vi "Ecrire config.vi"(2 "error in (no error)":errorcluster caption="entrée d'erreur (pas d'erreur)", 3 "refnum":T1) -> (0 "error out":errorcluster caption="sortie d'erreur", 1 "refnum out":T1 caption="refnum en sortie")   [LabVIEW 2022 SP3]
uses:
  <vilib>/Utility/config.llb/Config Data RefNum.ctl
  Variables globales/Variable glob Pt.vi
  <vilib>/Utility/config.llb/Write Key (Boolean).vi
  <vilib>/Utility/config.llb/Write Key (String).vi
  <vilib>/Utility/config.llb/Write Key (U32).vi
  <vilib>/Utility/config.llb/NI_LVConfig.lvlib
panel:
  out "Nb modules":u8
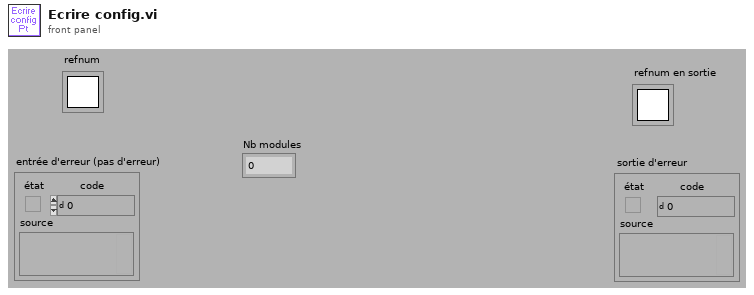
[diagram p1: front panel]
types:
  T1 = typedef "NI_LVConfig.lvlib/Config Data RefNum.ctl" = refnum<k1>
  T2 = cluster{"Nom tache Pt":refnum<k21>, "Noms des Pt":string[], "Nb Pt":i16, "Selection Pt":bool[], "Nom Pt selectionnees":string[]}[]
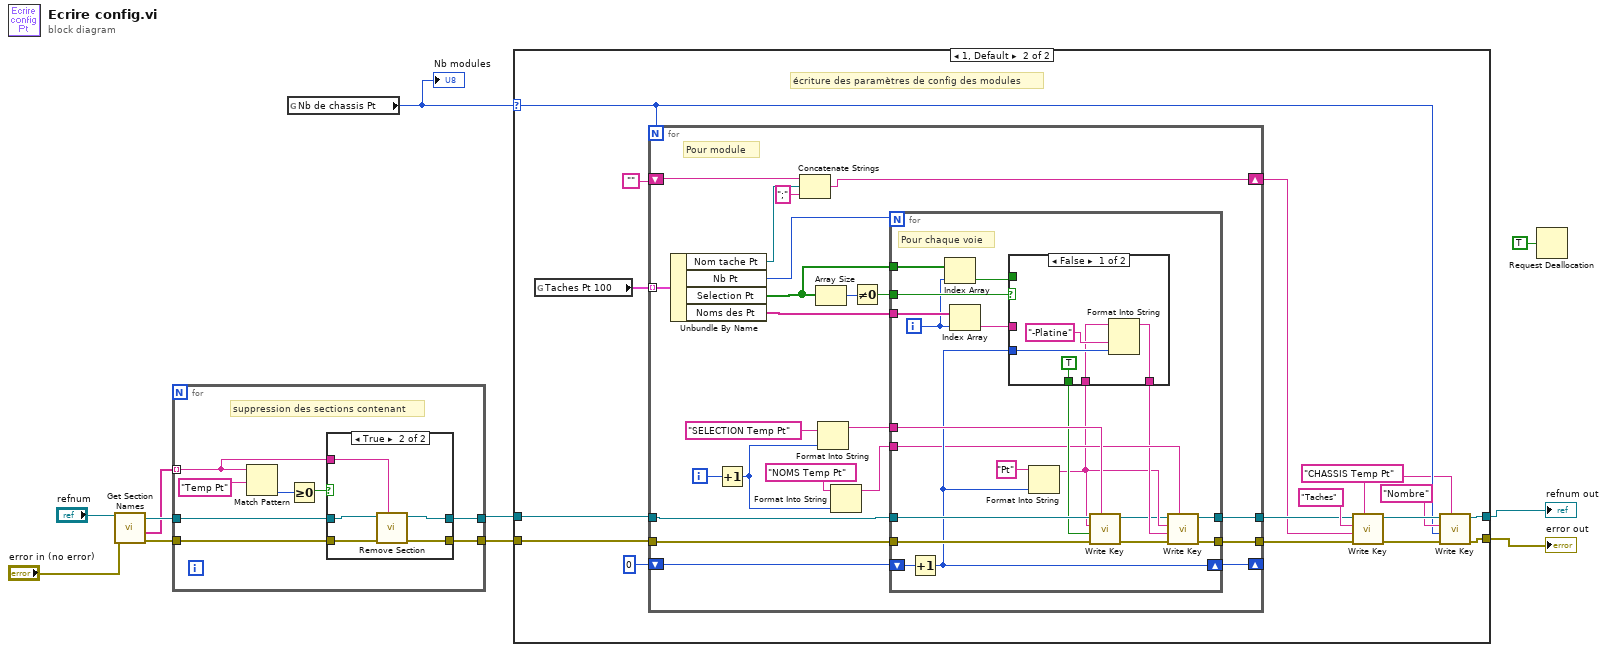
[diagram p0: block diagram]
diagram:
  n1 = call <vilib>:"Get Section Names.vi"("error in (no error)"="error in (no error)", "refnum"="refnum") -> ("error out"=w2:errorcluster, "section names"=w1:string[], "refnum out"=w3:T1)  [unwired: 7 in]
  n2 = for {
    tunnel: w1 -> [w16] mode=indexing
    tunnel: w2 -> [w14]
    tunnel: [w12] -> w4
    tunnel: w3 -> [w15]
    tunnel: [w13] -> w5
    # "suppression des sections contenant"
    n3 = Match Pattern(string=w16, regular expression="Temp Pt" ("expression régulière")) -> (offset past match=w18:i32)  [unwired: 1 in, 3 out]
    n4 = Greater Or Equal To 0?(x=w18) -> (x >= 0?=w17:bool)
    n5 = case shown="True" w17 {
      tunnel: w16 -> [_ w26]
      tunnel: w15 -> [w21 w24]
      tunnel: w14 -> [w20 w25]
      tunnel: [w21 w23] -> w13
      tunnel: [w20 w22] -> w12
      frame False {
      }
      frame True {
        n6 = call <vilib>:"Remove Section.vi"("section"=w26, "error in (no error)"=w25, "refnum"=w24) -> ("error out"=w22:errorcluster, "refnum out"=w23:T1)  [unwired: 6 in, 1 out]
      }
    }
  }
  n7 = global read "Variable glob Pt.vi" "Nb de chassis Pt"() -> (w7:u8)
  "Nb modules" <- w7
  n8 = case shown="1, Default" w7 {
    selector: w7 -> [_ w40]
    tunnel: w5 -> [w28 w35]
    tunnel: w4 -> [w27 w34]
    tunnel: [w28 w31] -> w10
    tunnel: [w27 w30] -> w11
    frame 0 {
      # "Pas de Pt"
    }
    frame 1, Default {
      w38 = "CHASSIS Temp Pt" ("section")
      # "écriture des paramètres de config des modules"
      n9 = global read "Variable glob Pt.vi" "Taches Pt 100"() -> (w37:T2)
      n10 = for {
        N: w40 -> [_]
        tunnel: [w63] -> w33
        tunnel: [w62] -> w32
        tunnel: w35 -> [w58]
        tunnel: w34 -> [w57]
        shift-right: [w55] -> _
        shift-left: 0 -> [w56]
        tunnel: w37 -> [w52] mode=indexing
        shift-right: [w45] -> w29
        shift-left: "" -> [w46]
        i -> [w54]
        # "Pour module"
        n11 = Unbundle By Name(w52) -> ("Nom tache Pt"=w48:refnum<k21>, "Nb Pt"=w51:i16, "Selection Pt"=w49:bool[], "Noms des Pt"=w50:string[])
        n12 = Increment(x=w54) -> (x+1=w53:i32)
        n13 = Concatenate Strings(w46, w48, ";" ("chaîne")) -> (w45:string)
        n14 = Array Size(array=w49) -> (size(s)=w60:i32)
        n15 = Format Into String(initial string="SELECTION Temp Pt" ("chaîne initiale"), w53) -> (resulting string=w64:string)  [unwired: 2 in, 1 out]
        n16 = Format Into String(initial string="NOMS Temp Pt", w53) -> (resulting string=w66:string)  [unwired: 2 in, 1 out]
        n17 = Not Equal To 0?(x=w60) -> (x != 0?=w59:bool)
        n18 = for {
          N: w51 -> [_]
          tunnel: w66 -> [w72]
          tunnel: w64 -> [w85]
          tunnel: w49 -> [w78]
          tunnel: w50 -> [w76]
          tunnel: w59 -> [w80]
          shift-right: [w73] -> w55
          shift-left: w56 -> [w74]
          tunnel: w57 -> [w83]
          tunnel: [w81] -> w62
          tunnel: w58 -> [w84]
          tunnel: [w82] -> w63
          i -> [w70]
          # "Pour chaque voie"
          n19 = Increment(x=w74) -> (x+1=w73:i32)
          n20 = Index Array(array=w78, index=w70) -> (element=w77:bool)
          n21 = Index Array(array=w76, index=w70) -> (element=w75:string)
          n22 = Format Into String(initial string="Pt", w73) -> (resulting string=w69:string)  [unwired: 2 in, 1 out]
          n23 = case shown="False" w80 {
            tunnel: w77 -> [_ w93]
            tunnel: w75 -> [_ w92]
            tunnel: [TRUE w93] -> w79
            tunnel: [w90 w92] -> w71
            tunnel: w73 -> [w89 _]
            tunnel: w69 -> [w87 _]
            frame False {
              n24 = Format Into String(initial string=w87, "-Platine" ("chaîne initiale"), w89) -> (resulting string=w90:string)  [unwired: 2 in, 1 out]
            }
            frame True {
            }
          }
          n25 = call-poly <vilib>:"Write Key.vi"("section"=w85, "error in (no error)"=w83, "value"=w79, "key"=w69, "refnum"=w84) -> ("error out"=w67:errorcluster, "refnum out"=w68:T1)  [unwired: 4 in, 1 out]
          n26 = call-poly <vilib>:"Write Key.vi"("section"=w72, "error in (no error)"=w67, "value"=w71, "key"=w69, "refnum"=w68) -> ("error out"=w81:errorcluster, "refnum out"=w82:T1)  [unwired: 4 in, 1 out]
        }
      }
      n27 = call-poly <vilib>:"Write Key.vi"("section"=w38, "error in (no error)"=w32, "value"=w29, "key"="Taches", "refnum"=w33) -> ("error out"=w42:errorcluster, "refnum out"=w43:T1)  [unwired: 4 in, 1 out]
      n28 = call-poly <vilib>:"Write Key.vi"("section"=w38, "error in (no error)"=w42, "value"=w40, "key"="Nombre", "refnum"=w43) -> ("error out"=w30:errorcluster, "refnum out"=w31:T1)  [unwired: 4 in, 1 out]
    }
  }
  "refnum out" <- w10
  "error out" <- w11
  n29 = Request Deallocation(TRUE ("flag")) -> ()
